vi "VIH Project Tree - Shortcut Menu Handler_(Add Expand Options).vi"(10 "Ena Expand/Collapse":bool, 11 "Menu dscr":string) -> (3 "Menu dscr out":string)   [LabVIEW 2014]
doc: "::: VI Helpeks :::\nCopyright (c) 2000-2026 Konstantin Shifershteyn. All rights reserved."
panel:
  # "VI Helpeks\nCopyright (c) 2012-2026 Konstantin Shifershteyn"
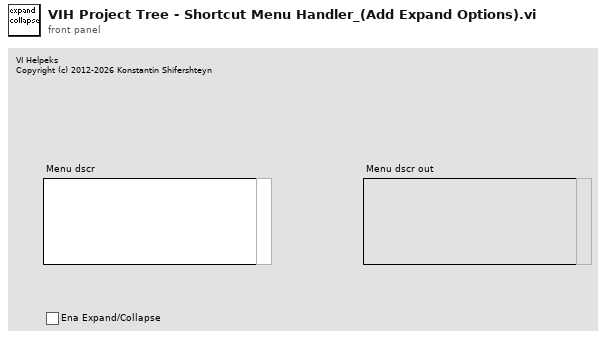
[diagram p1: front panel]
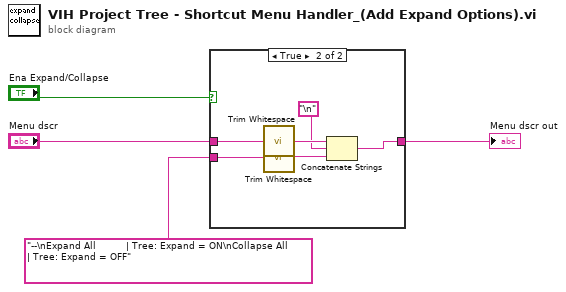
[diagram p0: block diagram]
diagram:
  n1 = case shown="True" "Ena Expand/Collapse" {
    tunnel: [w5 w9] -> w3
    tunnel: "Menu dscr" -> [w5 w11]
    tunnel: "--\nExpand All          | Tree: Expand = ON\nCollapse All        | Tree: Expand = OFF" -> [_ w6]
    frame False {
    }
    frame True {
      n2 = call <vilib>:"Trim Whitespace.vi"("string"=w11) -> ("trimmed string"=w10:string)  [unwired: 1 in]
      n3 = call <vilib>:"Trim Whitespace.vi"("string"=w6) -> ("trimmed string"=w7:string)  [unwired: 1 in]
      n4 = Concatenate Strings(w10, "\n", w7) -> (w9:string)
    }
  }
  "Menu dscr out" <- w3
